vi "Sim_Clock.vi"(2 "advance_ms":i64, 3 "current_ms":i64) -> (0 "valid":bool, 1 "next_ms":i64)   [LabVIEW 2026]
doc: "INTENT: Deterministic pure virtual-clock step. The caller owns the clock state. Accept only nonnegative current and increment with signed 64-bit overflow protection. On invalid input keep current_ms and set valid false. Synthetic only; never use as a hardware clock.. INPUTS: current_ms (int64), advance_ms (int64). OUTPUTS: next_ms (int64), valid (bool). DESIGN CONSTRAINT: Pure step: caller stores next_ms only when valid is true. Simulation-only virtual time; no wall clock or physical I/O. Signed 64-bit overflow and negative times are refused. REQUIREMENTS: SRS-F-006, A01-SIM-002. No physical hardware side effects. Acceptance requires native LabVIEW compilation and behavioral testing."
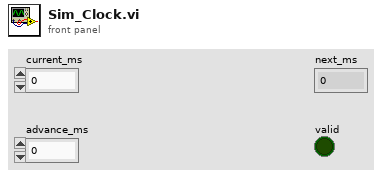
[diagram p1: front panel]
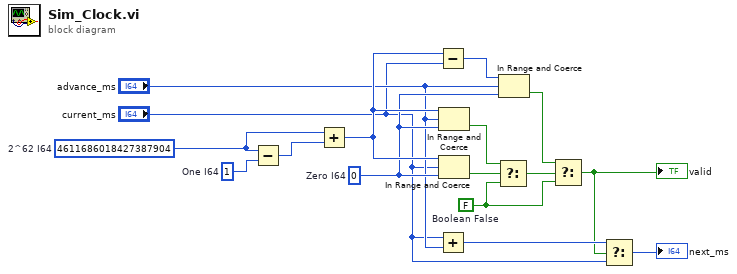
[diagram p0: block diagram]
diagram:
  w12 = FALSE  # Boolean False
  w5 = i64 1  # One I64
  w4 = i64 4611686018427387904  # 2^62 I64
  w3 = i64 0  # Zero I64
  n1 = Subtract(x=w4, y=w5) -> (x-y=w6:i64)
  n2 = Add(x=w4, y=w6) -> (x+y=w7:i64)
  n3 = Subtract(x=w7, y="current_ms") -> (x-y=w10:i64)
  n4 = Add(x="current_ms", y="advance_ms") -> (x+y=w15:i64)
  n5 = In Range and Coerce(upper limit=w7, x="advance_ms", lower limit=w3) -> (In Range?=w9:bool)  [unwired: 1 out]
  n6 = In Range and Coerce(upper limit=w7, x="current_ms", lower limit=w3) -> (In Range?=w8:bool)  [unwired: 1 out]
  n7 = Select(t=w9, s=w8, f=w12) -> (s? t:f=w13:bool)
  n8 = In Range and Coerce(upper limit=w10, x="advance_ms", lower limit=w3) -> (In Range?=w11:bool)  [unwired: 1 out]
  n9 = Select(t=w11, s=w13, f=w12) -> (s? t:f=w14:bool)
  "valid" <- w14
  n10 = Select(t=w15, s=w14, f="current_ms") -> (s? t:f=→"next_ms":i64)
